vi "Send and read from TCP Server.vi"(6 "timeout (ms)":i32=1000, 8 "error in (no error)":errorcluster, 10 "Message":string, 11 "IP Address":string) -> (0 "error out":errorcluster, 3 "Reply":string)   [LabVIEW 2020, in "TALOS.lvlib"]
uses:
  TALOS.lvlib
  Ancestor/Ancestor/Ancestor.lvclass/Ancestor.ctl
  Generate Error.vi
  FGV/Error Memory/Get Error Description.vi
  Get PC name.vi
  Ancestor/Ancestor/Read ID.vi
  Get Class Name.vi
  <vilib>/Utility/error.llb/Clear Errors.vi
  FGV/Error Memory/Error Memory Core.vi
  <vilib>/AdvancedString/Delimited String to 1D String Array.vi
  Circus Root Path.vi
  FGV/Error Memory/Error Crt Lvl checker.vi
  FGV/Error Memory/Error Memory Core.vi/40c8088d-b597-4017-91af-faa98e00292e.vi
  FGV/Error Memory/Error Memory Core.vi/d4a3ab98-063c-4e44-b43d-fbdcfe6c2be2.vi
  Global Memory.vi
  <vilib>/Utility/LVClass/Get LV Class Name.vi
  Is in Packed Library.vi
  TALOS Root path.vi
  Read CSV worksheet.vi
  <vilib>/Utility/error.llb/General Error Handler.vi
  Error Log.vi
  Ancestor/Ancestor/Ancestor.lvclass
  <vilib>/Comparison/Equal/Equal Functor/Equal Functor.lvclass
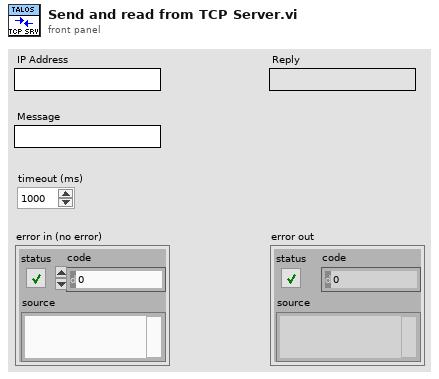
[diagram p1: front panel]
types:
  T1 = enum16{"Standard", "Buffered", "CRLF", "Immediate"}
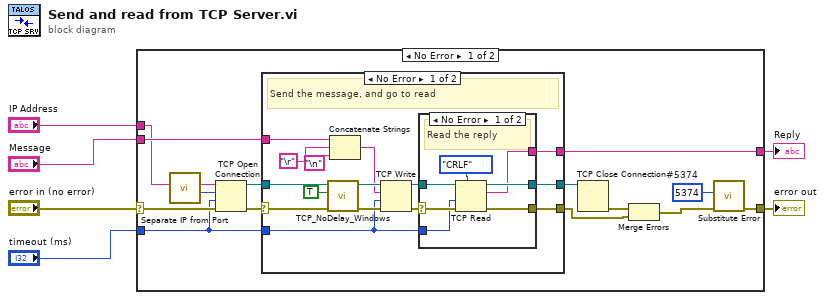
[diagram p0: block diagram]
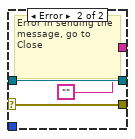
[diagram p2: hidden frame]
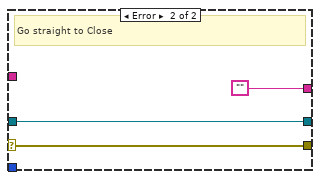
[diagram p3: hidden frame]
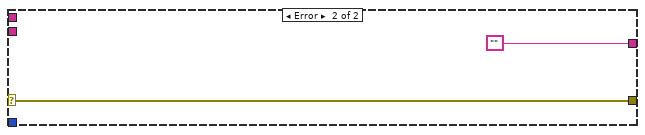
[diagram p4: hidden frame]
diagram:
  n1 = case shown="No Error" "error in (no error)" {
    selector: "error in (no error)" -> [w16 w51]
    tunnel: "Message" -> [w17 _]
    tunnel: "IP Address" -> [w7 _]
    tunnel: [w13 w51] -> w3
    tunnel: [w11 ""] -> w2
    tunnel: "timeout (ms)" -> [w10 _]
    frame No Error {
      w12 = 5374  # #5374
      n2 = call "Separate IP from Port.vi"("IP+Port"=w7) -> ("Port"=w8:u16, "IP"=w9:string)  [unwired: 9 in]
      n3 = TCP Open Connection(address=w9, remote port or service name=w8, timeout ms (60000)=w10, error in (no error)=w16) -> (connection ID=w18:refnum<k5>, error out=w19:errorcluster)  [unwired: 1 in]
      n4 = case shown="No Error" w19 {
        selector: w19 -> [w36 w49]
        tunnel: w10 -> [w25 _]
        tunnel: [w24 w48] -> w20
        tunnel: w18 -> [w33 w48]
        tunnel: w17 -> [w28 _]
        tunnel: [w23 w49] -> w15
        tunnel: [w22 ""] -> w11
        frame No Error {
          # "Send the message, and go to read"
          n5 = call "TCP_NoDelay_Windows.vi"("error in (no error)"=w36, "TCP_NODELAY (true)"=TRUE, "connID"=w33) -> ("error out"=w35:errorcluster, "connID 2"=w34:refnum<k5>)  [unwired: 3 in]
          n6 = Concatenate Strings(w28, "\r", "\n") -> (w29:string)
          n7 = TCP Write(connection ID=w34, data in=w29, error in (no error)=w35, 9:w25) -> (connection ID out=w26:refnum<k5>, error out=w27:errorcluster)  [unwired: 1 out]
          n8 = case shown="No Error" w27 {
            selector: w27 -> [w42 w45]
            tunnel: w26 -> [w43 w46]
            tunnel: w25 -> [w41 _]
            tunnel: [w39 w46] -> w24
            tunnel: [w38 w45] -> w23
            tunnel: [w37 ""] -> w22
            frame No Error {
              # "Read the reply"
              n9 = TCP Read(connection ID=w43, error in (no error)=w42, 7:T1."CRLF" ("mode (standard)"), 9:w41) -> (connection ID out=w39:refnum<k5>, data out=w37:string, error out=w38:errorcluster)  [unwired: 1 in]
            }
            frame Error {
              # "Error in sending the message, go to Close"
            }
          }
        }
        frame Error {
          # "Go straight to Close"
        }
      }
      n10 = TCP Close Connection(connection ID=w20) -> (error out=w21:errorcluster)  [unwired: 2 in, 1 out]
      n11 = Merge Errors(w21, w15) -> (w14:errorcluster)
      n12 = call "Substitute Error.vi"("error in (no error)"=w14, "Error Code"=w12) -> ("error out"=w13:errorcluster)  [unwired: 9 in]
    }
    frame Error {
    }
  }
  "error out" <- w3
  "Reply" <- w2
